vi "TCP Error Handle.vi"(8 "错误输入（无错误）":errorcluster) -> (0 "错误输出":errorcluster, 3 "Stop?":bool)   [LabVIEW 2020, in "TCP Communication.lvlib"]
uses:
  TCP Communication.lvlib
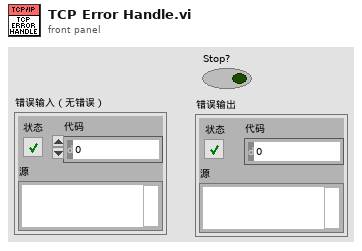
[diagram p1: front panel]
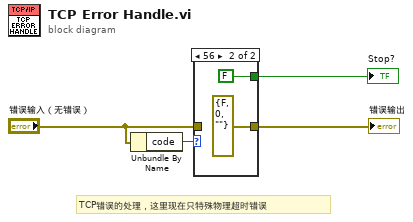
[diagram p0: block diagram]
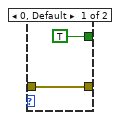
[diagram p2: hidden frame]
diagram:
  # "TCP错误的处理，这里现在只特殊物理超时错误"
  n1 = Unbundle By Name("错误输入（无错误）") -> ("code"=w3:i32)
  n2 = case shown="56" w3 {
    tunnel: [TRUE FALSE] -> w4
    tunnel: [w5 errorcluster {"status"=FALSE, "code"=0, "source"=""} ("错误输入（无错误）")] -> w1
    tunnel: "错误输入（无错误）" -> [w5 _]
    frame 0, Default {
    }
    frame 56 {
    }
  }
  "Stop?" <- w4
  "错误输出" <- w1
